vi "BuildSpecifications.vi"(6 "ItemBuilt":T3, 8 "error in (no error)":errorcluster, 11 "SolutionBuilder in":refnum<class "SolutionBuilder.lvclass">) -> (0 "error out":errorcluster, 1 "Generated file":T1, 3 "SolutionBuilder out":refnum<class "SolutionBuilder.lvclass">)   [LabVIEW 2019, in "SolutionBuilder.lvlib" / "SolutionBuilder.lvclass"]
uses:
  SolutionBuilder.lvclass
  Events/EventItemBuilt.ctl
  BuildManager/GeneratedFile.ctl
  BuildManager/BuildProjectInfo.ctl
  SolutionBuilder.lvclass/SolutionBuilder.ctl
  BuildManager/BuildManager.lvclass
  BuildManager/BuildManager.lvclass/BuildManager.ctl
  SolutionBuilder.lvlib
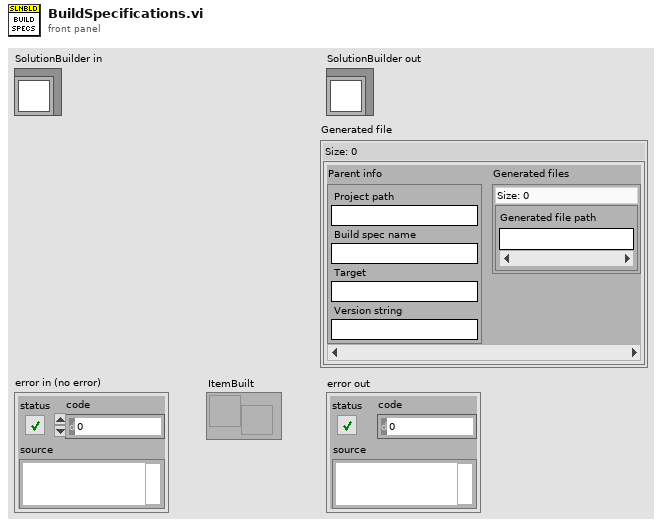
[diagram p1: front panel]
types:
  T1 = typedef "SolutionBuilder.lvlib/BuildManager.lvclass/GeneratedFile.ctl" = map{T2, set{string}}
  T2 = typedef "SolutionBuilder.lvlib/BuildManager.lvclass/BuildProjectInfo.ctl" = cluster{"Project path":string, "Build spec name":string, "Target":string, "Version string":string}
  T3 = typedef "SolutionBuilder.lvlib/EventItemBuilt.ctl" = refnum<user-event>
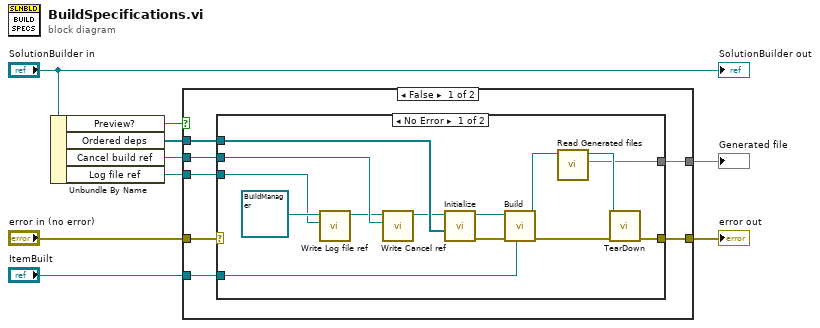
[diagram p0: block diagram]
diagram:
  n1 = Unbundle By Name("SolutionBuilder in") -> ("Preview?"=w7:bool, "Ordered deps"=w9:refnum<class "ProjectItem.lvclass">[], "Cancel build ref"=w2:refnum<vi>, "Log file ref"=w1:refnum<file>)
  n2 = case shown="False" w7 {
    tunnel: w9 -> [w16 _]
    tunnel: "ItemBuilt" -> [w15 _]
    tunnel: "error in (no error)" -> [w14 w32]
    tunnel: [w13 w32] -> w5
    tunnel: [w12 _] -> w4
    tunnel: w2 -> [w11 _]
    tunnel: w1 -> [w10 _]
    frame False {
      n3 = case shown="No Error" w14 {
        selector: w14 -> [_ w31]
        tunnel: w16 -> [w30 _]
        tunnel: w15 -> [w28 _]
        tunnel: [w25 w31] -> w13
        tunnel: [w22 _] -> w12
        tunnel: w11 -> [w20 _]
        tunnel: w10 -> [w17 _]
        frame No Error {
          n4 = call "Write Log file ref.vi"("Log file ref"=w17, "BuildManager in"=refnum<class "BuildManager.lvclass"> refnum ("SolutionBuilder.lvlib:BuildManager.lvclass")) -> ("BuildManager out"=w18:refnum<class "BuildManager.lvclass">)  [unwired: 9 in]
          n5 = call "Write Cancel ref.vi"("Cancel build ref"=w20, "BuildManager in"=w18) -> ("BuildManager out"=w21:refnum<class "BuildManager.lvclass">)  [unwired: 9 in]
          n6 = call "Initialize.vi"("Ordered deps"=w30, "BuildManager in"=w21) -> ("error out"=w26:errorcluster, "BuildManager out"=w29:refnum<class "BuildManager.lvclass">)  [unwired: 8 in]
          n7 = call "Build.vi"("ItemBuilt"=w28, "error in (no error)"=w26, "BuildManager in"=w29) -> ("error out"=w27:errorcluster, "BuildManager out"=w24:refnum<class "BuildManager.lvclass">)  [unwired: 7 in]
          n8 = call "Read Generated files.vi"("BuildManager in"=w24) -> ("Generated file"=w22:T1, "BuildManager out"=w23:refnum<class "BuildManager.lvclass">)  [unwired: 9 in]
          n9 = call "TearDown.vi"("error in (no error)"=w27, "BuildManager in"=w23) -> ("error out"=w25:errorcluster)  [unwired: 8 in, 1 out]
        }
        frame Error {
        }
      }
    }
    frame True {
    }
  }
  "error out" <- w5
  "Generated file" <- w4
  "SolutionBuilder out" <- "SolutionBuilder in"
